vi "CreateDbCommand.vi"(8 "error in (no error)":errorcluster, 11 "DbConnection in":refnum<class "ORM_DBC_dotNetCore.lvclass">) -> (0 "error out":errorcluster, 2 "Command":refnum<k39>, 3 "DbConnection out":refnum<class "ORM_DBC_dotNetCore.lvclass">)   [LabVIEW 2026, in "ORM_DBC_dotNetCore.lvlib" / "ORM_DBC_dotNetCore.lvclass"]
uses:
  ORM_DBC_dotNetCore.lvclass
  C:/Program Files/dotnet/shared/Microsoft.NETCore.App/8.0.28/System.Data.Common.dll
  Program Files/dotnet/shared/Microsoft.NETCore.App/8.0.28/System.Data.Common.dll
  ORM_DBC_dotNetCore.lvclass/ORM_DBC_dotNetCore.ctl
  Read connection.vi
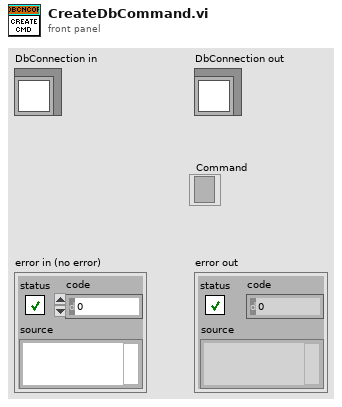
[diagram p1: front panel]
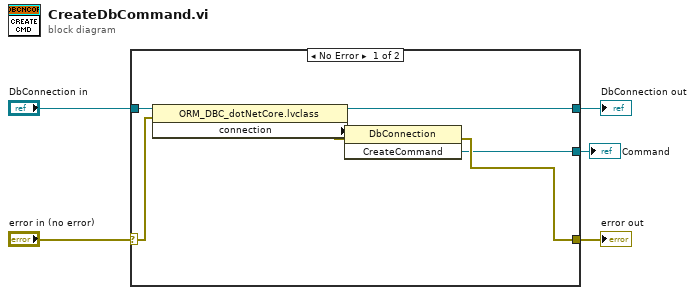
[diagram p0: block diagram]
diagram:
  n1 = case shown="No Error" "error in (no error)" {
    selector: "error in (no error)" -> [w9 w14]
    tunnel: [w7 w14] -> w4
    tunnel: [w10 w13] -> w2
    tunnel: "DbConnection in" -> [w11 w13]
    tunnel: [w6 _] -> w1
    frame No Error {
      n2 = property class="ORM_DBC_dotNetCore.lvclass"(reference=w11, error in=w9) -> (reference out=w10:refnum<class "ORM_DBC_dotNetCore.lvclass">, error out=w8:errorcluster, "connection"=w12:refnum<k39>)
      n3 = invoke class="DbConnection" method="CreateCommand"(reference=w12, error in=w8) -> (error out=w7:errorcluster, "CreateCommand"=w6:refnum<k39>)  [unwired: 1 in, 1 out]
    }
    frame Error {
    }
  }
  "error out" <- w4
  "DbConnection out" <- w2
  "Command" <- w1
